vi "ISP Exmpl - Echo Generator.vi"() -> ()   [LabVIEW 2021]
doc: "::: CalcExpress Toolkit :::\nCopyright (c) 2000-2026 Konstantin Shifershteyn. All rights reserved."
panel:
  in  "GenRequest":string="Generate"
  in  "stop":bool
  in  "decay":dbl=35.0 format="%.2f"
  in  "echo amplitude":dbl=0.3 format="%.2f"
  in  "echo delay":i32=117
  in  "amplitude":dbl=1.0 format="%.2f"
  out "Signal":dbl[](graph)=[1.0, 0.9632527198929306, 0.8696386802901347, 0.7255262217165931, 0.540203056136529, 0.3252823630066793, 0.09397863442544156, -0.13970178052493915, -0.3618060270148575, -0.5592651359152437, -0.7206601994731159, -0.8368795863948778, -0.901629565190355, -0.9117699608235621, -0.8674572872221521, -0.7720895109002396, -0.6320584986851149, -0.4563275740121081, -0.25586178142272104, -0.04294684832078443, 0.1695610381565001, 0.36900898670477195, 0.5436982714451026, 0.6835679068646907, 0.780771146483551, 0.8301120559310516, 0.8293181036265088, 0.7791348153178652, 0.6832393322757534, 0.5479805444063637, 0.38196369320414464, 0.19550635478187353, 2.4461386135839145e-16, -0.1927835230126453, -0.3713985057849455, -0.5254026293959191, -0.645965012865096, -0.7263698039021738, -0.76238676917117, -0.7524886612469677, -0.6979045482139943, -0.6025082137576444, -0.4725505724599948, -0.3162542120596283, -0.14329613494146132, 0.035788932297249304, 0.21024801160205864, 0.3697534409214423, 0.5050121436498081, 0.6083047850762379, 0.6739236761144389, 0.6984847496444397, 0.68109677962031, 0.6233797511780877, 0.5293333883681992, 0.40506575785073556, 0.25840006368145735, 0.0983847518759479, -0.06526254679716044, -0.22274319142479018, -0.3647623395763458, -0.4830756012483521, -0.5709655067094342, -0.6236203837417246, -0.6383944346660991, -0.6149351755566301, -0.5551724936675938, -0.4631719021481959, -0.3448626246271787, -0.20765845023850157, -0.059995437194722945, 0.08918483920006536, 0.2309749540749372, 0.3570317502710714, 0.4600654606289973, 0.5342592704401566, 0.5755952965479374, 0.5820688686854892, 0.553779904473174, 0.49289764682278364, 0.4035026279439872, 0.2913169836340135, 0.16334073730401982, 0.02741702895443823, -0.1082468230953159, -0.2355732834541019, -0.3470939506281309, -0.4363859474587727, -0.4984399546629688, -0.529938916655617, -0.5294320619230065, -0.4973953299535242, -0.4361761872698223, -0.34982772985432237, -0.24384349598603555, -0.12481016883460382, -1.3745547640000495e-15, 0.1230719281865963, 0.23709873913641394, 0.3354141145652901, 0.4123804692020918, 0.4637104403206535, 0.4867034705019428, 0.48038457348940755, 0.4455383795079727, 0.38463789050349284, 0.3016736555567401, 0.20189492891857855, 0.09147945505579236, -0.022847455201205485, -0.13422116050636743, -0.23604853888288949, -0.3223969419448338, -0.38833838937342774, -0.43022912422117665, -0.4459087768721539, -0.43480839357860857, -0.097962163835629, -0.048947673249327694, 0.00229987860132419, 0.0526967039433697, 0.09925263878734822, 0.13924795556944736, 0.17039160409298315, 0.19095171340384304, 0.19985096725547025, 0.19672166109503922, 0.18191772248311902, 0.15648357829418497, 0.12208232419866671, 0.08088804199002353, 0.03544917845847395, -0.0114684729837356, -0.057049550661887743, -0.09859751899316158, -0.1336936394287301, -0.1603371797249329, -0.17705877092519728, -0.18300053363621632, -0.17795866348423547, -0.16238646187677874, -0.1373581824161435, -0.10449639226628296, -0.06586768350372837, -0.02385338745722762, 0.018996658607056516, 0.06011834567276657, 0.0970862292616505, 0.12775607586889604, 0.1503886731131191, 0.16374778948347485, 0.1671668084886888, 0.1605805042532863, 0.14452055124639876, 0.1200755406947927, 0.08881837971988693, 0.05270585211284323, 0.01395671136667595, -0.02508413336028273, -0.0620870545642498, -0.09487626361788856, -0.12155727450038711, -0.14062583584185995, -0.15105210056632085, -0.15233536422717728, -0.1445265213023294, -0.12821735137824494, -0.10449773538075405, -0.07488379701470985, -0.041221654773045346, -0.0055728574393753005, 0.02991141750153134, 0.0631197523613151, 0.09210570735117068, 0.11520146744447439, 0.1311133094947518, 0.13899345606351496, 0.13848436467028905, 0.12973319815956308, 0.11337602951112011, 0.09049314348417323, 0.06253850020051466, 0.031247922192225552, -0.0014682296994930621, -0.033641282522695215, -0.06336233222776763, -0.08889511987416622, -0.10877705176679085, -0.12190251112696941, -0.12758374525852834, -0.1255860136213433, -0.11613526160035537, -0.09989824549964466, -0.07793667633953133, -0.05163847583746889, -0.0226305582413745, 0.007321409326936007, 0.0364201156427498, 0.06294410739712046, 0.08534927536155669, 0.10235836320645443, 0.1130333339674662, 0.1168265222142865, 0.11360782036895359, 0.1036666135272544, 0.08768869921031686, 0.0667099152654804, 0.042049562573128724, 0.015227869800628957, -0.012127361131997208, -0.03837921729882619, -0.06197930844335381, -0.08155876782948376, -0.09600729195223397, -0.10453567749512692, -0.10671836020007301, -0.10251370023117339, -0.09226111561057804, -0.07665555691907852, -0.056701159309236526, -0.033647122663173296, -0.008909886862727534, 0.016013571135627375, 0.03963603009862817, 0.06056847867557275, 0.07760148753422738, 0.08977475097171246, 0.09643082034616264, 0.09725004872546335, 0.09226492686105829, 0.08185324354749919, 0.06671077270228398, 0.047805399260856946, 0.026315674994839083, 0.003557681174484295, -0.019095282465950922, -0.04029529862496673, -0.058799770973971065, -0.07354397568191959, -0.08370200709210367, -0.08873264880595466, -0.08840764769378275, -0.0828209516964995, -0.07237862626443849, -0.05777031917573695, -0.03992423048037308, -0.01994849962239656, 0.0009373096689683363, 0.021476407537517922, 0.04045016026167096, 0.05675014979664403, 0.06944266446730486, 0.07782188467527959, 0.08144875292690221, 0.08017341216776656, 0.07414010467415828]
  in  "cycles":dbl=10.0 format="%.2f"
  in  "samples":i32=256
  in  "generate":bool
  in  "Notifier":string="COMM_Notifier"
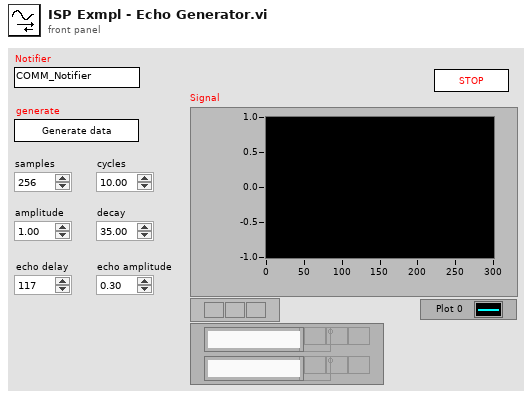
[diagram p1: front panel]
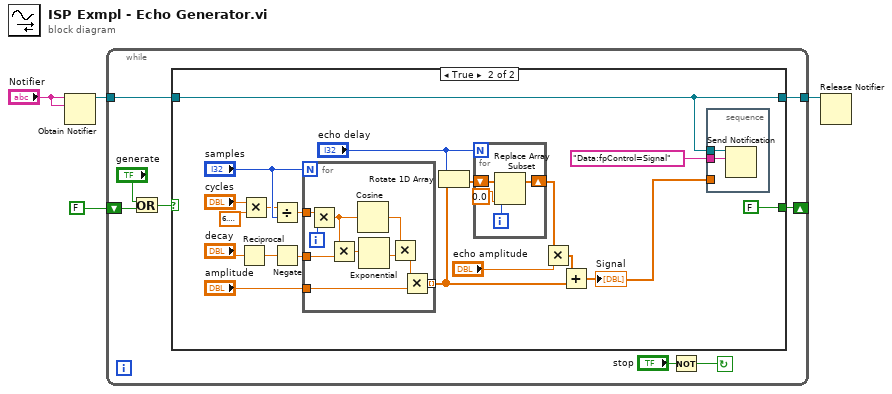
[diagram p0: block diagram]
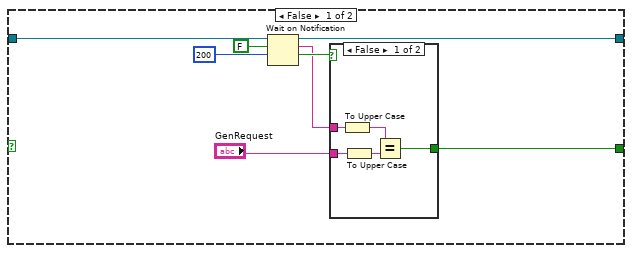
[diagram p2: hidden frame]
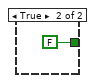
[diagram p3: hidden frame]
diagram:
  n1 = Obtain Notifier(name (unnamed)="Notifier", notification data type="Notifier") -> (notifier out=w4:refnum<notifier>)  [unwired: 2 in, 2 out]
  n2 = while {
    shift-left: FALSE -> [w7]
    shift-right: [w8] -> _
    tunnel: [w9] -> w3
    tunnel: w4 -> [w10]
    stop <- w11 continue-if-true
    n3 = Or(x="generate", y=w7) -> (x .or. y?=w5:bool)
    n4 = case shown="True" w5 {
      tunnel: w10 -> [w20 w29]
      tunnel: [w19 w29] -> w9
      tunnel: [w13 FALSE] -> w8
      frame False {
        n5 = Wait on Notification(notifier=w20, ignore previous (F)=FALSE ("ignore previous (T)"), timeout in ms (-1)=200 ("ms timeout (-1)")) -> (notifier out=w19:refnum<notifier>, notification=w15:string, timed out?=w16:bool)  [unwired: 1 in, 1 out]
        n6 = case shown="False" w16 {
          tunnel: w15 -> [w24 _]
          tunnel: "GenRequest" -> [w25 _]
          tunnel: [w21 FALSE] -> w13
          frame False {
            n7 = To Upper Case(1:w24) -> (0:w23:string)
            n8 = To Upper Case(1:w25) -> (0:w22:string)
            n9 = Equal?(x=w23, y=w22) -> (x = y?=w21:bool)
          }
          frame True {
          }
        }
      }
      frame True {
        n10 = Reciprocal(x="decay") -> (1/x=w33:dbl)
        n11 = Multiply(x="cycles", y=6.283185307179586) -> (x*y=w41:dbl)
        n12 = Divide(x=w41, y="samples") -> (x/y=w44:dbl)
        n13 = Negate(x=w33) -> (-x=w35:dbl)
        n14 = for {
          N: "samples" -> [_]
          tunnel: w44 -> [w60]
          tunnel: "amplitude" -> [w59]
          tunnel: [w58] -> w32 mode=indexing
          tunnel: w35 -> [w55]
          i -> [w61]
          n15 = Multiply(x=w60, y=w61) -> (x*y=w56:dbl)
          n16 = Multiply(x=w56, y=w55) -> (x*y=w57:dbl)
          n17 = Cosine(x=w56) -> (cos(x)=w53:dbl)
          n18 = Exponential(1:w57) -> (0:w54:dbl)
          n19 = Multiply(x=w53, y=w54) -> (x*y=w52:dbl)
          n20 = Multiply(x=w52, y=w59) -> (x*y=w58:dbl)
        }
        n21 = Rotate 1D Array(1:w32, 2:"echo delay") -> (0:w38:dbl[])
        n22 = for {
          N: "echo delay" -> [_]
          shift-right: [w49] -> w36
          shift-left: w38 -> [w50]
          i -> [w51]
          n23 = Replace Array Subset(array=w50, new element=0.0, index=w51) -> (w49:dbl[])
        }
        n24 = Multiply(x=w36, y="echo amplitude") -> (x*y=w31:dbl[])
        n25 = Add(x=w31, y=w32) -> (x+y=w27:dbl[])
        "Signal" <- w27
        n26 = stacked-sequence {
          tunnel: "Data:fpControl=Signal" -> [w47]
          tunnel: w29 -> [w46]
          tunnel: w27 -> [_]
          frame #0 {
            n27 = Send Notification(notification=w47, notifier=w46) -> ()  [unwired: 1 in, 2 out]
          }
        }
      }
    }
    n28 = Not(x="stop") -> (.not. x?=w11:bool)
  }
  n29 = Release Notifier(notifier=w3) -> ()  [unwired: 2 in, 3 out]
